vi "Init.vi"(8 "error in (no error)":errorcluster, 11 "uService Template in":refnum<class "TCP Text Listener.lvclass">) -> (0 "error out":errorcluster, 3 "uService Template out":refnum<class "TCP Text Listener.lvclass">)   [LabVIEW 2020, in "TALOS.lvlib" / "TCP Text Listener.lvlib" / "TCP Text Listener.lvclass"]
uses:
  TCP Text Listener.lvclass
  C:/LabVIEW Code/TALOS/talos/Internal uServices/System uServices/TCP Listener/TCP Listener/TCP Listener.lvclass
  TCP Text Listener.lvclass/TCP Text Listener.ctl
  TCP Listener/TCP Listener/TCP Listener.lvclass
  Father of all uServices/Father of all uServices/Father of all uServices.lvclass
  C:/LabVIEW Code/TALOS/talos/Father of all uServices/Father of all uServices/Father of all uServices.lvclass
  C:/LabVIEW Code/TALOS/talos/Ancestor/Ancestor/Ancestor.lvclass
  C:/LabVIEW Code/TALOS/builds/Actor Framework PPL/Actor Framework.lvlibp/1abvi3w/vi.lib/ActorFramework/Actor/Actor.lvclass
  C:/LabVIEW Code/TALOS/talos/Internal uServices/System uServices/TCP Text Listener/TCP Text Listener.lvclass
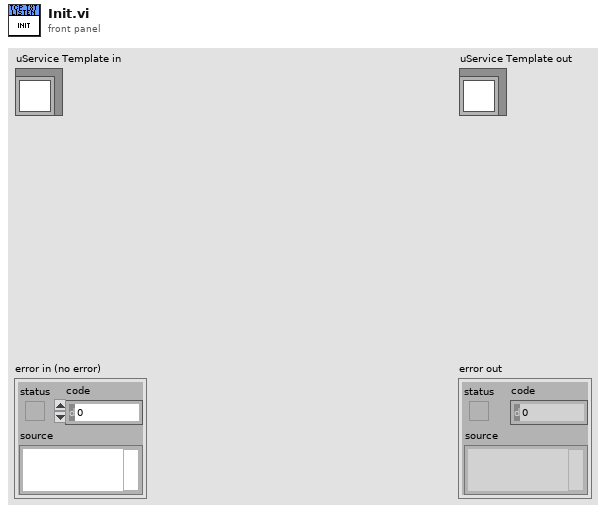
[diagram p1: front panel]
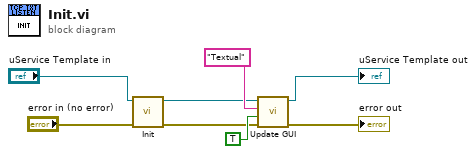
[diagram p0: block diagram]
diagram:
  n1 = call-parent "Init.vi"("error in (no error)"="error in (no error)", "uService Template in"="uService Template in") -> ("error out"=w3:errorcluster, "uService Template out"=w4:refnum<class "TCP Text Listener.lvclass">)  [unwired: 8 in]
  n2 = call "Update GUI.vi"("error in (no error)"=w3, "Data"=TRUE ("Textual"), "GUI Item Name"="Textual", "uService Template in"=w4) -> ("error out"=→"error out":errorcluster, "uService Template out"=→"uService Template out":refnum<class "TCP Text Listener.lvclass">)  [unwired: 6 in]
